vi "Invalid project element extension--error.vi"() -> (0 "error out":errorcluster)   [LabVIEW 2026]
doc: "Invalid extension. This error is triggered when a project item with an invalid extension (i.e. not .ctl or .vi) is added to a project item."
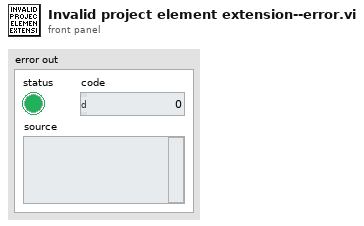
[diagram p1: front panel]
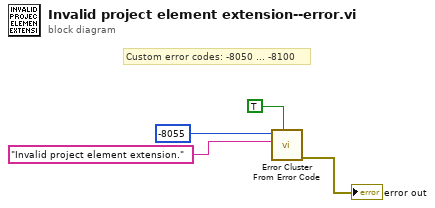
[diagram p0: block diagram]
diagram:
  # "Custom error codes: -8050 ... -8100"
  n1 = call <vilib>:"Error Cluster From Error Code.vi"("show call chain? (False)"=TRUE, "error message (\"\")"="Invalid project element extension." ("error message (\"\")"), "error code (0)"=-8055) -> ("error out"=→"error out":errorcluster)  [unwired: 6 in]
